vi "Test Helper Loop Restart.vi"(8 "error in (no error)":errorcluster, 11 "Helper Loop Test In":refnum<class "Helper Loop Test.lvclass">) -> (0 "error out":errorcluster, 3 "Helper Loop Test Out":refnum<class "Helper Loop Test.lvclass">)   [LabVIEW 2020, in "Helper Loop Test.lvclass"]
uses:
  Helper Loop Test.lvclass
  C:/Program Files (x86)/National Instruments/LabVIEW 2020/vi.lib/Astemes/LUnit/Test Case.lvclass
  source/Framework Test Suite/Mock Process/Mock Process.lvclass
  C:/git/astemes-triarc-framework/source/Framework/Process/Process.lvclass
  <vilib>/Astemes/LUnit/Test Case.lvclass/Test Case.ctl
  source/Framework/Process/Process.lvclass/Process.ctl
  5c824806-a2a3-41ed-ad4d-6f7d99db2d3e.vi
  f58b967f-3bde-4b6b-a42a-cab2bdf802bc.vi
  source/Framework/Broadcast Event Dequeuers/Execution timer.vi
  <vilib>/Astemes/LUnit/Append Pass Result.vi
  <vilib>/Astemes/LUnit/Append Fail Result.vi
  5c824806-a2a3-41ed-ad4d-6f7d99db2d3e.vi/9c5d11cd-9439-4240-a1ee-d9baace9c924.vi
  source/Framework/Process/Private/SubVIs/Wait for finish.vi
  source/Framework/Process/Private/SubVIs/Set Lifecycle State.vi
  source/Framework/Process/Protected/Messaging/Send Message.vi
  f58b967f-3bde-4b6b-a42a-cab2bdf802bc.vi/9c5d11cd-9439-4240-a1ee-d9baace9c924.vi
  <vilib>/Astemes/LUnit/Run In UI.vi
  source/Framework/Process/Private/SubVIs/Handle Debug Data.vi
  <vilib>/Utility/error.llb/Clear Errors.vi
  source/Framework/Logging/Log Debug.vi
  <vilib>/AdvancedString/1D String Array to Delimited String.vi
  <vilib>/Utility/High Resolution Relative Seconds.vi
  source/Framework/Broadcast Event Dequeuers/Dequeue Broadcast Message.vi
  source/Framework/Process/Public/Lifecycle/Get Lifecycle State.vi
  <vilib>/Utility/error.llb/Error Cluster From Error Code.vi
  source/Framework/Process/Public/Read Name.vi
  source/Framework/Callback/Callback.lvclass
  source/Framework/Process/Process.lvclass
  Helper Loop Test.lvclass/Helper Loop Test.ctl
  source/Framework/Broadcast Event Dequeuers/Broadcast Event Dequeuers.lvlib
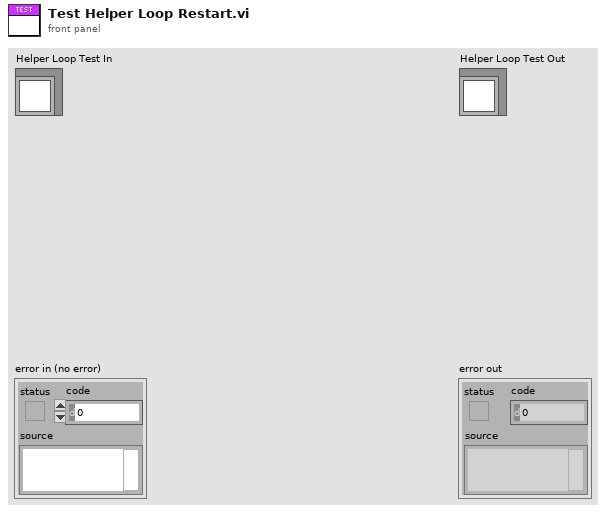
[diagram p1: front panel]
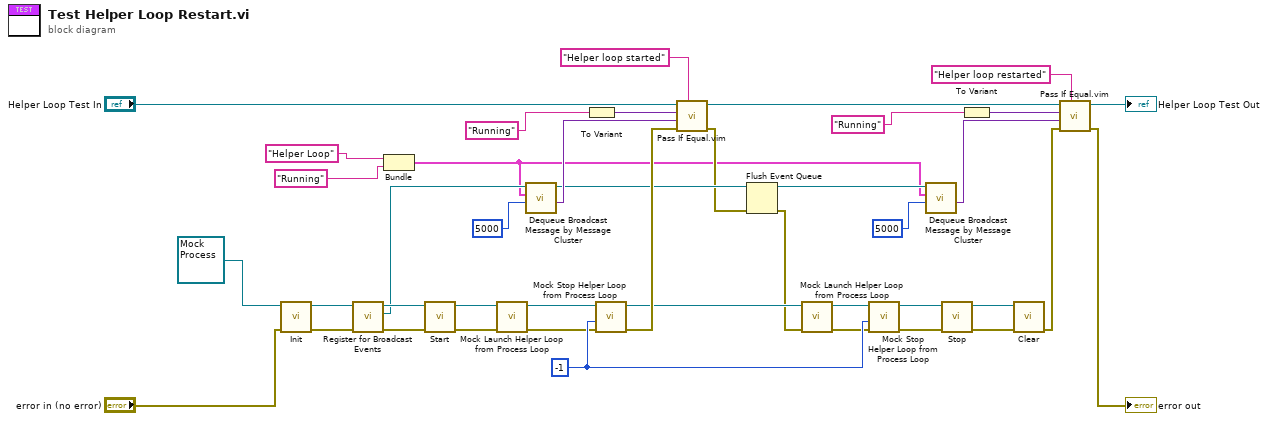
[diagram p0: block diagram]
diagram:
  w25 = -1 ("timeout in ms (-1)")
  n1 = call-dynamic "Init.vi"("error in (no error)"="error in (no error)", "Mock Process In"=refnum<class "Mock Process.lvclass"> refnum) -> ("error out"=w42:errorcluster, "Mock Process Out"=w22:refnum<class "Mock Process.lvclass">)  [unwired: 8 in]
  n2 = call "Register for Broadcast Events.vi"("error in (no error)"=w42, "Process In"=w22) -> ("error out"=w23:errorcluster, "Event Registration Refnum Out"=w15:refnum<event-registration>, "Process Out"=w21:refnum<class "Mock Process.lvclass">)  [unwired: 7 in]
  n3 = Bundle("y"="Helper Loop", "Description"="Running") -> (w3:cluster{"y":string, "Description":string})  [unwired: 1 in]
  n4 = call "Start.vi"("error in (no error)"=w23, "Process In"=w21) -> ("error out"=w40:errorcluster, "Process Out"=w41:refnum<class "Mock Process.lvclass">)  [unwired: 7 in, 1 out]
  n5 = call "Mock Launch Helper Loop from Process Loop.vi"("error in (no error)"=w40, "Mock Process in"=w41) -> ("error out"=w18:errorcluster, "Mock Process out"=w19:refnum<class "Mock Process.lvclass">)  [unwired: 8 in]
  n6 = call "Dequeue Broadcast Message by Message Cluster.vi"("Timeout (-1)"=5000, "Message"=w3, "Event Registration Refnum"=w15) -> ("Message Data"=w14:variant, "Event Registration Refnum Out"=w10:refnum<event-registration>)  [unwired: 4 in, 3 out]
  n7 = To Variant(anything="Running") -> (Variant=w2:variant)
  n8 = call "Mock Stop Helper Loop from Process Loop.vi"("error in (no error)"=w18, "timeout in ms (-1)"=w25, "Mock Process in"=w19) -> ("error out"=w29:errorcluster, "Mock Process out"=w28:refnum<class "Mock Process.lvclass">)  [unwired: 6 in, 1 out]
  n9 = call "Pass If Equal.vim"("Description"="Helper loop started", "error in (no error)"=w29, "Actual"=w14, "Expected"=w2, "LUnit Test Case In"="Helper Loop Test In") -> ("error out"=w9:errorcluster, "LUnit Test Case Out"=w31:refnum<class "Helper Loop Test.lvclass">)  [unwired: 5 in]
  n10 = Flush Event Queue(0:w10, 3:w9) -> (8:w11:refnum<event-registration>, 11:w8:errorcluster)  [unwired: 4 in, 1 out]
  n11 = call "Mock Launch Helper Loop from Process Loop.vi"("error in (no error)"=w8, "Mock Process in"=w28) -> ("error out"=w16:errorcluster, "Mock Process out"=w17:refnum<class "Mock Process.lvclass">)  [unwired: 8 in]
  n12 = call "Mock Stop Helper Loop from Process Loop.vi"("error in (no error)"=w16, "timeout in ms (-1)"=w25, "Mock Process in"=w17) -> ("error out"=w26:errorcluster, "Mock Process out"=w27:refnum<class "Mock Process.lvclass">)  [unwired: 6 in, 1 out]
  n13 = call "Dequeue Broadcast Message by Message Cluster.vi"("Timeout (-1)"=5000, "Message"=w3, "Event Registration Refnum"=w11) -> ("Message Data"=w7:variant)  [unwired: 4 in, 4 out]
  n14 = call "Stop.vi"("error in (no error)"=w26, "Process In"=w27) -> ("error out"=w39:errorcluster, "Process Out"=w24:refnum<class "Mock Process.lvclass">)  [unwired: 7 in, 1 out]
  n15 = To Variant(anything="Running") -> (Variant=w1:variant)
  n16 = call-dynamic "Clear.vi"("error in (no error)"=w39, "Mock Process In"=w24) -> ("error out"=w38:errorcluster)  [unwired: 9 in]
  n17 = call "Pass If Equal.vim"("Description"="Helper loop restarted", "error in (no error)"=w38, "Actual"=w7, "Expected"=w1, "LUnit Test Case In"=w31) -> ("error out"=→"error out":errorcluster, "LUnit Test Case Out"=→"Helper Loop Test Out":refnum<class "Helper Loop Test.lvclass">)  [unwired: 5 in]
